vi "RemoteVI Mouse Captured.vi"(0 "hWnd":u64, 11 "error in":errorcluster) -> (4 "captured?":bool, 15 "error out":errorcluster)   [LabVIEW 2020, in "RemoteVI.lvlib"]
doc: "Tells whether the thread that owns hWnd (LabVIEW's UI thread) holds the mouse capture. LabVIEW captures the mouse while it TRACKS a press - a latched button, a slider, a text selection, a graph drag - and while tracking it reads the coordinates of posted moves and of the button-up as SCREEN coordinates; without capture they are CLIENT coordinates, as Windows defines them (measured: a switch that does not track lost its posted button-up when it carried screen coordinates, a latched button lost it with client coordinates). RemoteVI Translate Input.vi takes the answer as tracking in. Reads user32 GetWindowThreadProcessId.vi then user32 GetGUIThreadInfo.vi with the 64-bit GUITHREADINFO (cbSize 72, hwndCapture in info[6,7]); when that call fails it is repeated with the 32-bit layout (cbSize 48, hwndCapture in info[4]). Both calls run in any thread, so this answers even while a LabVIEW popup holds the UI thread. An incoming error skips the work and answers FALSE."
uses:
  RemoteVI.lvlib
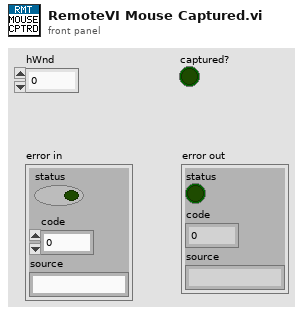
[diagram p1: front panel]
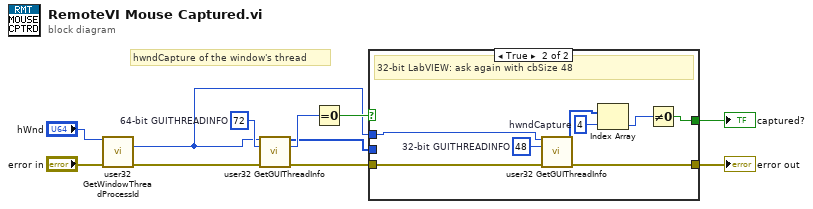
[diagram p0: block diagram]
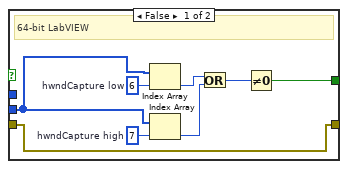
[diagram p2: hidden frame]
diagram:
  w5 = u32 72  # 64-bit GUITHREADINFO
  # "hwndCapture of the window's thread"
  n1 = call "user32 GetWindowThreadProcessId.vi"("hWnd"="hWnd", "error in"="error in") -> ("thread ID"=w3:u32, "error out"=w4:errorcluster)  [unwired: 11 in, 1 out]
  n2 = call "user32 GetGUIThreadInfo.vi"("thread ID"=w3, "cbSize"=w5, "error in"=w4) -> ("info"=w6:u32[], "return value"=w7:i32, "error out"=w8:errorcluster)  [unwired: 10 in]
  n3 = Equal To 0?(x=w7) -> (x = 0?=w9:bool)
  n4 = case shown="True" w9 {
    tunnel: w3 -> [_ w20]
    tunnel: w6 -> [w12 _]
    tunnel: w8 -> [w13 w21]
    tunnel: [w13 w24] -> w11
    tunnel: [w19 w27] -> w10
    frame False {
      w15 = 7  # hwndCapture high
      w14 = 6  # hwndCapture low
      # "64-bit LabVIEW"
      n5 = Index Array(array=w12, index=w14) -> (element=w16:u32)
      n6 = Index Array(array=w12, index=w15) -> (element=w17:u32)
      n7 = Or(x=w16, y=w17) -> (x .or. y?=w18:u32)
      n8 = Not Equal To 0?(x=w18) -> (x != 0?=w19:bool)
    }
    frame True {
      w25 = 4  # hwndCapture
      w22 = u32 48  # 32-bit GUITHREADINFO
      # "32-bit LabVIEW: ask again with cbSize 48"
      n9 = call "user32 GetGUIThreadInfo.vi"("thread ID"=w20, "cbSize"=w22, "error in"=w21) -> ("info"=w23:u32[], "error out"=w24:errorcluster)  [unwired: 10 in, 1 out]
      n10 = Index Array(array=w23, index=w25) -> (element=w26:u32)
      n11 = Not Equal To 0?(x=w26) -> (x != 0?=w27:bool)
    }
  }
  "captured?" <- w10
  "error out" <- w11
